vi "helper loop.vi"(11 "helper loop data":T1) -> ()   [LabVIEW 2025, in "XButton.lvlib" / "button3.xctl"]
uses:
  button3.xctl
  helper loop Events.ctl
  move event.ctl
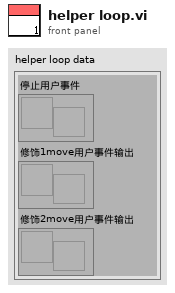
[diagram p1: front panel]
types:
  T1 = typedef "XButton.lvlib/button3.xctl/helper loop Events.ctl" = cluster{"停止用户事件":refnum<user-event>, "修饰1move用户事件输出":refnum<user-event>, "修饰2move用户事件输出":refnum<user-event>}
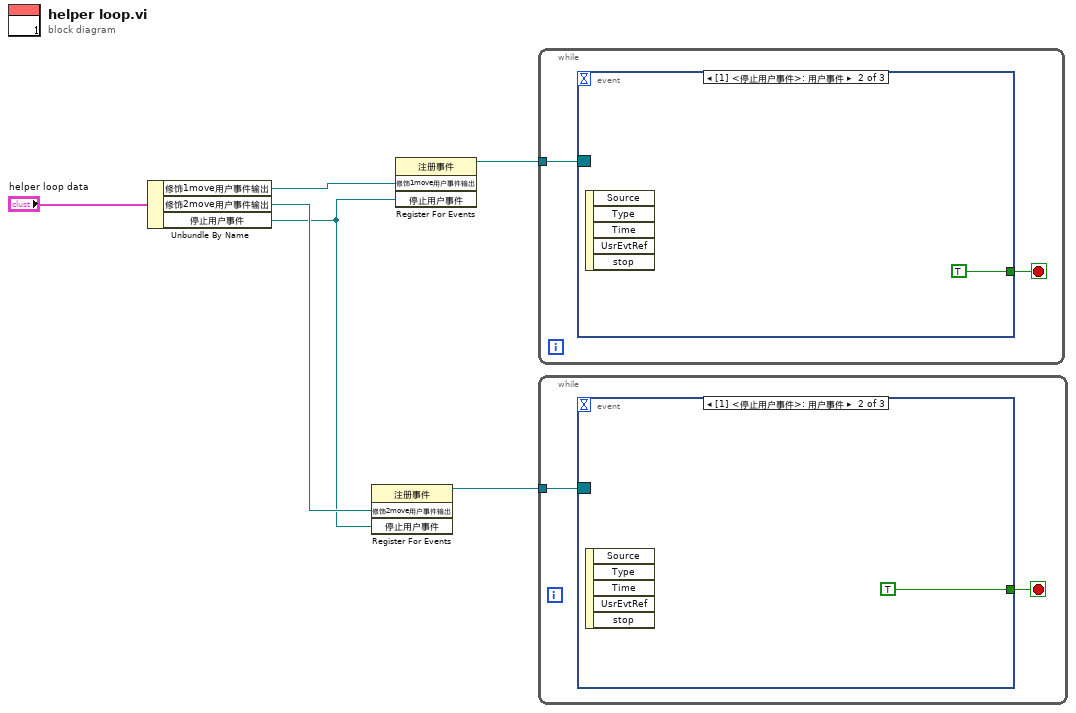
[diagram p0: block diagram]
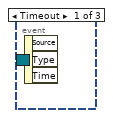
[diagram p2: hidden frame]
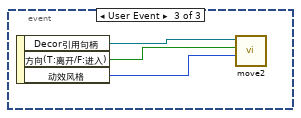
[diagram p3: hidden frame]
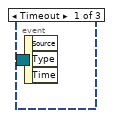
[diagram p4: hidden frame]
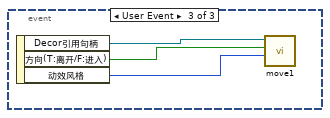
[diagram p5: hidden frame]
diagram:
  n1 = Unbundle By Name("helper loop data") -> ("修饰1move用户事件输出"=w4:refnum<user-event>, "修饰2move用户事件输出"=w3:refnum<user-event>, "停止用户事件"=w2:refnum<user-event>)
  n2 = register-events(w3, w2) -> (reference out=w1:refnum<event-registration>)  [unwired: 2 in, 1 out]
  n3 = register-events(w4, w2) -> (reference out=w6:refnum<event-registration>)  [unwired: 2 in, 1 out]
  n4 = while {
    tunnel: w6 -> [w7]
    stop <- w8 stop-if-true
    n5 = event shown="[1] <停止用户事件>: 用户事件" {
      selector: w7 -> [_ _ _]
      dyn-events: _ -> [_ _ _]
      timeout: _ -> [_ _ _]
      tunnel: [_ TRUE _] -> w8
      event Timeout {
        n6 = event-data() -> ()  [unwired: 1 in, 3 out]
      }
      event User Event {
        n7 = event-data() -> ()  [unwired: 1 in, 5 out]
      }
      event User Event {
        n8 = event-data() -> ("Decor引用句柄"=w12:refnum<vi>, "方向(T:离开/F:进入)"=w11:bool, "动效风格"=w10:enum16{"风格一", "风格二", "风格三", "风格四"})  [unwired: 1 in]
        n9 = call "move1.vi"("动效风格"=w10, "In(T)/Out(F)"=w11, "Decor引用句柄"=w12) -> ()  [unwired: 8 in, 1 out]
      }
    }
  }
  n10 = while {
    tunnel: w1 -> [w13]
    stop <- w14 stop-if-true
    n11 = event shown="[1] <停止用户事件>: 用户事件" {
      selector: w13 -> [_ _ _]
      dyn-events: _ -> [_ _ _]
      timeout: _ -> [_ _ _]
      tunnel: [_ TRUE _] -> w14
      event Timeout {
        n12 = event-data() -> ()  [unwired: 1 in, 3 out]
      }
      event User Event {
        n13 = event-data() -> ()  [unwired: 1 in, 5 out]
      }
      event User Event {
        n14 = event-data() -> ("Decor引用句柄"=w18:refnum<vi>, "方向(T:离开/F:进入)"=w17:bool, "动效风格"=w16:enum16{"风格一", "风格二", "风格三", "风格四"})  [unwired: 1 in]
        n15 = call "move2.vi"("动效风格"=w16, "In(T)/Out(F)"=w17, "Decor引用句柄"=w18) -> ()  [unwired: 8 in, 1 out]
      }
    }
  }
